vi "eDyno Vibration Stats.vi"(0 "Acceleration (g)":dbl[](array[numeric])) -> (4 "RMS (g)":dbl, 6 "Peak (g)":dbl, 8 "Crest Factor":dbl, 10 "Kurtosis":dbl)   [LabVIEW 2026]
doc: "Overall time-domain metrics of one acquired block (g): RMS, absolute Peak, Crest Factor = Peak/RMS, and Kurtosis = mean(x^4)/mean(x^2)^2 (about 3 for Gaussian noise; rises well above 3 with impulsive content such as a bearing defect). Assumes an AC (zero-mean) signal."
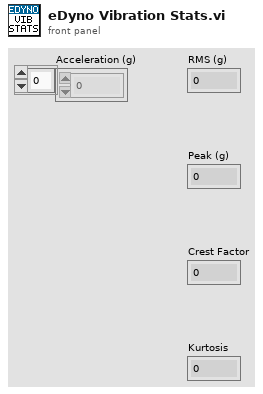
[diagram p1: front panel]
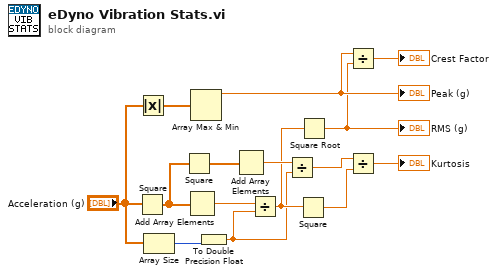
[diagram p0: block diagram]
diagram:
  n1 = Square(x="Acceleration (g)") -> (x^2=w6:dbl[])
  n2 = Absolute Value(x="Acceleration (g)") -> (abs(x)=w15:dbl[])
  n3 = Array Size(array="Acceleration (g)") -> (size(s)=w8:i32)
  n4 = Square(x=w6) -> (x^2=w11:dbl[])
  n5 = Add Array Elements(numeric array=w6) -> (sum=w7:dbl)
  n6 = Array Max & Min(array=w15) -> (max value=w3:dbl)  [unwired: 3 out]
  "Peak (g)" <- w3
  n7 = To Double Precision Float(number=w8) -> (double precision float=w9:dbl)
  n8 = Add Array Elements(numeric array=w11) -> (sum=w12:dbl)
  n9 = Divide(x=w7, y=w9) -> (x/y=w10:dbl)
  n10 = Divide(x=w12, y=w9) -> (x/y=w13:dbl)
  n11 = Square(x=w10) -> (x^2=w14:dbl)
  n12 = Square Root(x=w10) -> (sqrt(x)=w2:dbl)
  "RMS (g)" <- w2
  n13 = Divide(x=w3, y=w2) -> (x/y=→"Crest Factor":dbl)
  n14 = Divide(x=w13, y=w14) -> (x/y=→"Kurtosis":dbl)
